vi "Create CIF PCAP Config.vi"(11 "PCAP FIFO Config":T2 {"Linktype" items=["L2 Enet"=1, "SocketCAN"=227, "I2C_Linux"=209, "FlexRay"=210, "MOST"=211, "LIN"=212, "Universal"=0]}) -> (3 "Flattened PCAP FIFO Config":u8[](array[numeric]))   [LabVIEW 2021, in "Iceoryx Channel Utilities.lvlib"]
uses:
  Iceoryx Channel Utilities.lvlib
  ChannelCommon/ChannelCommon.lvlib
  <vilib>/CIF Foundation/CIF Utilities/DataTypes/DataTypes_CIF_U.lvlib
  ChannelCommon/typedef/FIFO Flags.ctl
  ChannelCommon/typedef/New FIFO Config.ctl
  Typedef/PCAP Linktype.ctl
  Typedef/PCAP Config.ctl
panel:
  in  "Linktype":T1=4294967295 items=["Universal"=4294967295, "L2 Enet"=1, "SocketCAN"=227, "I2C_Linux"=209, "FlexRay"=210, "MOST"=211, "LIN"=212, "CIF_Telemetry"=150, "CIF_DAQ_Waveform"=151]
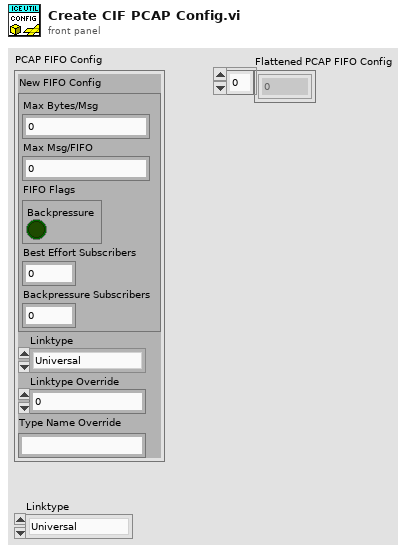
[diagram p1: front panel]
types:
  T1 = typedef "Iceoryx Channel Utilities.lvlib/PCAP Linktype.ctl" = u32
  T2 = typedef "Iceoryx Channel Utilities.lvlib/PCAP Config.ctl" = cluster{"New FIFO Config":T3, "Linktype":T1, "Linktype Override":u32, "Type Name Override":string}
  T3 = typedef "ChannelCommon.lvlib/New FIFO Config.ctl" = cluster{"Max Bytes/Msg":u64, "Max Msg/FIFO":u64, "FIFO Flags":T4, "Best Effort Subscribers":u32, "Backpressure Subscribers":u32}
  T4 = typedef "ChannelCommon.lvlib/FIFO Flags.ctl" = cluster{"Backpressure":bool, "Extended Config":bool}
  T5 = typedef "LVStringsAndValuesArrayTypeDef_U32.ctl" = cluster{"String":string, "Value":u32}[]
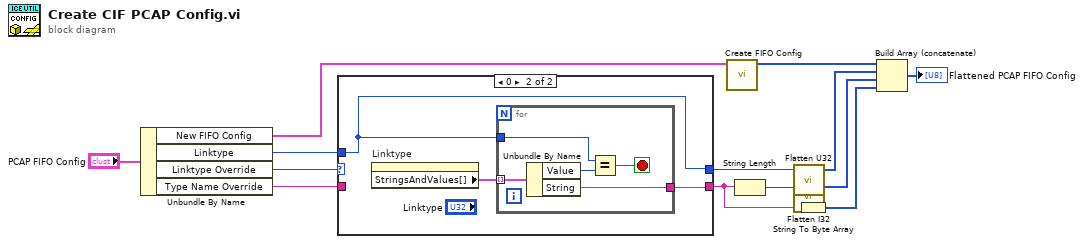
[diagram p0: block diagram]
diagram:
  n1 = Unbundle By Name("PCAP FIFO Config") -> ("New FIFO Config"=w12:T3, "Linktype"=w10:T1, "Linktype Override"=w11:u32, "Type Name Override"=w9:string)
  n2 = case shown="0" w11 {
    selector: w11 -> [w14 _]
    tunnel: w10 -> [_ w16]
    tunnel: w9 -> [w15 _]
    tunnel: [w15 w17] -> w6
    tunnel: [w14 w16] -> w7
    frame 1, Default {
    }
    frame 0 {
      n3 = property on="Linktype" class="Ring (strict)"() -> ("StringsAndValues[]"=w18:T5)  [unwired: 2 in, 2 out]
      n4 = for {
        tunnel: w18 -> [w23] mode=indexing
        tunnel: w16 -> [w21]
        tunnel: [w19] -> w17
        stop <- w20 stop-if-true
        n5 = Unbundle By Name(w23) -> ("Value"=w22:u32, "String"=w19:string)
        n6 = Equal?(x=w21, y=w22) -> (x = y?=w20:bool)
      }
    }
  }
  n7 = call "Create FIFO Config.vi"("New FIFO Config"=w12) -> ("Flattened FIFO Config"=w5:u8[])  [unwired: 10 in]
  n8 = String Length(string=w6) -> (length=w8:i32)
  n9 = call <vilib>:"Flatten U32.vi"("U32"=w7) -> ("Flat Data"=w4:u8[])  [unwired: 4 in]
  n10 = call <vilib>:"Flatten I32.vi"("I32"=w8) -> ("Flat Data"=w3:u8[])  [unwired: 4 in]
  n11 = String To Byte Array(string=w6) -> (unsigned byte array=w2:u8[])
  n12 = Build Array (concatenate)(w5, w4, w3, w2) -> (→"Flattened PCAP FIFO Config":u8[])
